vi "Copy .LLB to NI VeriStand dir.vi"(5 "Files Generated by Build":path[](array[path]), 6 "Top Level/Always Included VIs":path[](array[path]), 7 "Destination Path":path, 8 "error in (no error)":errorcluster, 9 "Target Name":string, 10 "Build Specification Name":string, 11 "Project Path":path) -> (0 "error out":errorcluster)   [LabVIEW 2024]
doc: "This VI is called after each run of a build specification. The VI will copy the generated LLB (Engine or System Explorer) into the VeriStand Custom Device folder (...\\Documents\\National Instruments\\NI VeriStand 2013...)."
uses:
  <vilib>/Utility/sysdir.llb/System Directory Type.ctl
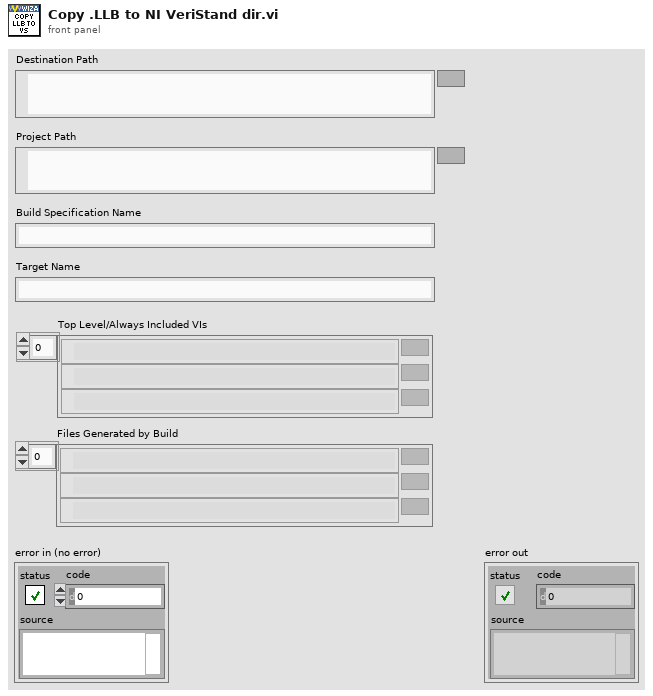
[diagram p1: front panel]
types:
  T1 = typedef "System Directory Type.ctl" = i32
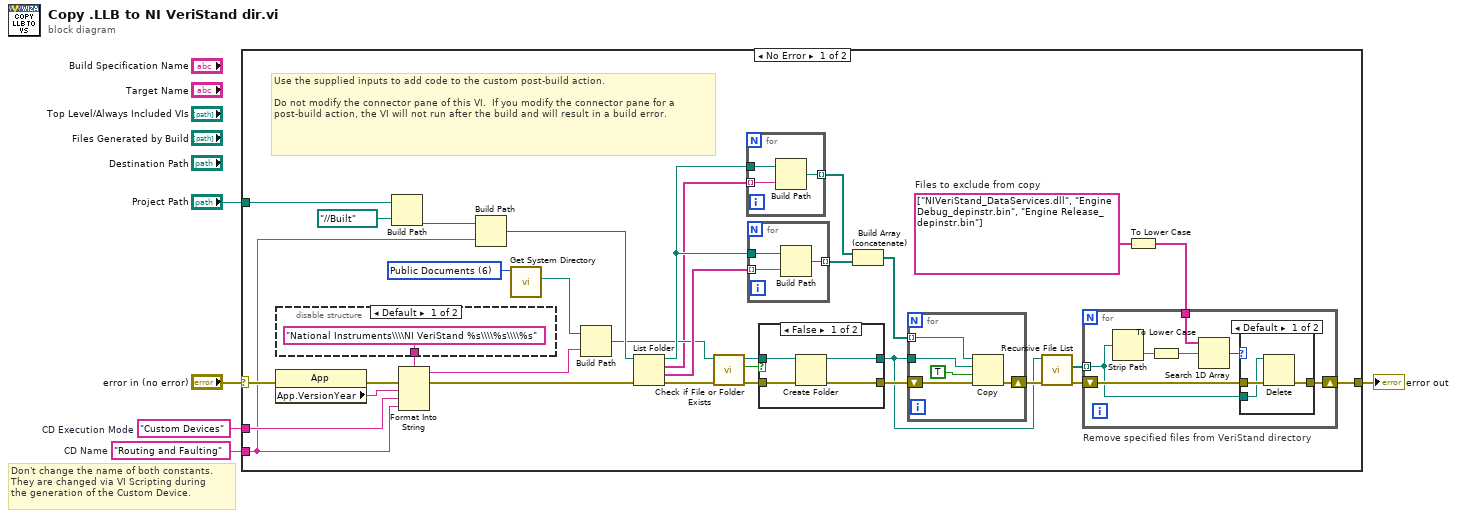
[diagram p0: block diagram]
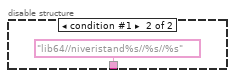
[diagram p2: hidden frame]
diagram:
  w2 = "Routing and Faulting"  # CD Name
  w3 = "Custom Devices"  # CD Execution Mode
  # "Don't change the name of both constants.\nThey are changed via VI Scripting during\nthe generation of the Custom Device."
  n1 = case shown="No Error" "error in (no error)" {
    selector: "error in (no error)" -> [w19 w69]
    tunnel: [w6 w69] -> w1
    tunnel: "Project Path" -> [w15 _]
    tunnel: w3 -> [w20 _]
    tunnel: w2 -> [w17 _]
    frame No Error {
      w12 = string[] ["NIVeriStand_DataServices.dll", "Engine Debug_depinstr.bin", "Engine Release_depinstr.bin"]  # Files to exclude from copy
      w25 = T1 6 items=["User Home"=0, "User Desktop"=1, "User Documents"=2, "User Application Data"=3, "User Preferences"=4, "User Temporary"=5, "Public Documents"=6, "Public Application Data"=7, "Public Preferences"=8, "Public Cache"=13, "System Core Libraries"=9, "System Installed Libraries"=10, "Application Files"=11, "Boot Volume Root"=12] ("system directory type")
      # "Use the supplied inputs to add code to the custom post-build action.\n\nDo not modify the connector pane of this VI.  If you modify the connector pane for a post-build action, the VI will not run after the build and will result in a build error."
      n2 = property class="App"(error in=w19) -> (error out=w24:errorcluster, "App.VersionYear"=w23:string)  [unwired: 1 in, 1 out]
      n3 = disable-structure shown="Default" {
        disable-tunnel: ["National Instruments\\\\NI VeriStand %s\\\\%s\\\\%s" ("name or relative path") "lib64//niveristand%s//%s//%s" ("name or relative path")] -> w22
        frame condition #0 (active) {
        }
        frame condition #1 {
        }
      }
      n4 = Build Path(base path=w15, name or relative path=path "../../Built") -> (appended path=w28:path)
      n5 = Format Into String(format string=w22, error in=w24, w23, w20, w17) -> (resulting string=w27:string, error out=w18:errorcluster)  [unwired: 1 in]
      n6 = Build Path(base path=w28, name or relative path=w17) -> (appended path=w30:path)
      n7 = call <vilib>:"Get System Directory.vi"("system directory type"=w25) -> ("system directory"=w26:path)  [unwired: 10 in]
      n8 = Build Path(base path=w26, name or relative path=w27) -> (appended path=w21:path)
      n9 = List Folder(path=w30, error in=w18) -> (path out=w32:path, filenames=w13:string[], folder names=w33:string[], error out=w29:errorcluster)  [unwired: 2 in]
      n10 = call <vilib>:"Check if File or Folder Exists.vi"("error in (no error)"=w29, "path"=w21) -> ("error out"=w34:errorcluster, "file or folder exists?"=w36:bool, "dup path"=w35:path)  [unwired: 7 in]
      n11 = for {
        tunnel: w13 -> [w67] mode=indexing
        tunnel: w32 -> [w68]
        tunnel: [w66] -> w38 mode=indexing
        n12 = Build Path(base path=w68, name or relative path=w67) -> (appended path=w66:path)
      }
      n13 = for {
        tunnel: w33 -> [w64] mode=indexing
        tunnel: w32 -> [w65]
        tunnel: [w63] -> w31 mode=indexing
        n14 = Build Path(base path=w65, name or relative path=w64) -> (appended path=w63:path)
      }
      n15 = case shown="False" w36 {
        tunnel: w35 -> [w55 w57]
        tunnel: w34 -> [w54 w56]
        tunnel: [w53 w57] -> w7
        tunnel: [w52 w56] -> w14
        frame False {
          n16 = Create Folder(path (use dialog)=w55, error in=w54) -> (created path=w53:path, error out=w52:errorcluster)  [unwired: 1 in, 1 out]
        }
        frame True {
        }
      }
      n17 = Build Array (concatenate)(w38, w31) -> (w37:path[])
      n18 = for {
        tunnel: w37 -> [w59] mode=indexing
        shift-right: [w60] -> w8
        shift-left: w14 -> [w61]
        tunnel: w7 -> [w58]
        n19 = Copy(8:w61, 9:TRUE ("overwrite (F)"), 10:w58, 11:w59) -> (0:w60:errorcluster)  [unwired: 1 in, 2 out]
      }
      n20 = call <vilib>:"Recursive File List.vi"("error in (no error)"=w8, "Folder Path"=w7) -> ("error out"=w11:errorcluster, "All Files in Dir"=w10:path[])  [unwired: 5 in, 3 out]
      n21 = To Lower Case(string=w12) -> (all lower case string=w9:string[])
      n22 = for "Remove specified files from VeriStand directory" {
        shift-right: [w42] -> w6
        shift-left: w11 -> [w44]
        tunnel: w10 -> [w41] mode=indexing
        tunnel: w9 -> [w45]
        n23 = Strip Path(path=w41) -> (name=w47:string)  [unwired: 1 out]
        n24 = To Lower Case(string=w47) -> (all lower case string=w46:string)
        n25 = Search 1D Array(1D array=w45, element=w46) -> (index of element=w43:i32)  [unwired: 1 in]
        n26 = case shown="Default" w43 {
          tunnel: w44 -> [w50 w51]
          tunnel: [w49 w51] -> w42
          tunnel: w41 -> [w48 _]
          frame Default {
            n27 = Delete(path (use dialog)=w48, error in=w50) -> (error out=w49:errorcluster)  [unwired: 3 in, 2 out]
          }
          frame -1 {
          }
        }
      }
    }
    frame Error {
    }
  }
  "error out" <- w1
